vi "identify new classes.vi"(7 "existing progress bar?":bool, 8 "error in":errorcluster, 10 "force scan":bool, 11 "cache in":T1) -> (0 "error out":errorcluster, 3 "cache out":T1)   [LabVIEW 2013, in "PL_class cache.lvlib"]
uses:
  PL_class cache.lvlib
  cache definition.ctl
  cache search configuration.ctl
  cached class information.ctl
  target class metadata.ctl
  class metadata.ctl
  <vilib>/NI/Tag Bus Module Framework/root configuration/Target Types.ctl
  <vilib>/NI/Configuration Framework/class discovery singleton/class discovery singleton methods.ctl
  <vilib>/NI/Progress Bar/Controls/Update Bar Actions.ctl
  cache data.vi
  <vilib>/NI/Configuration Framework/class discovery singleton/class discovery singleton.lvlib
  <vilib>/NI/Tag Bus Module Framework/root configuration/TBM configuration.lvclass
  <vilib>/NI/Progress Bar/Progress Bar.lvlib
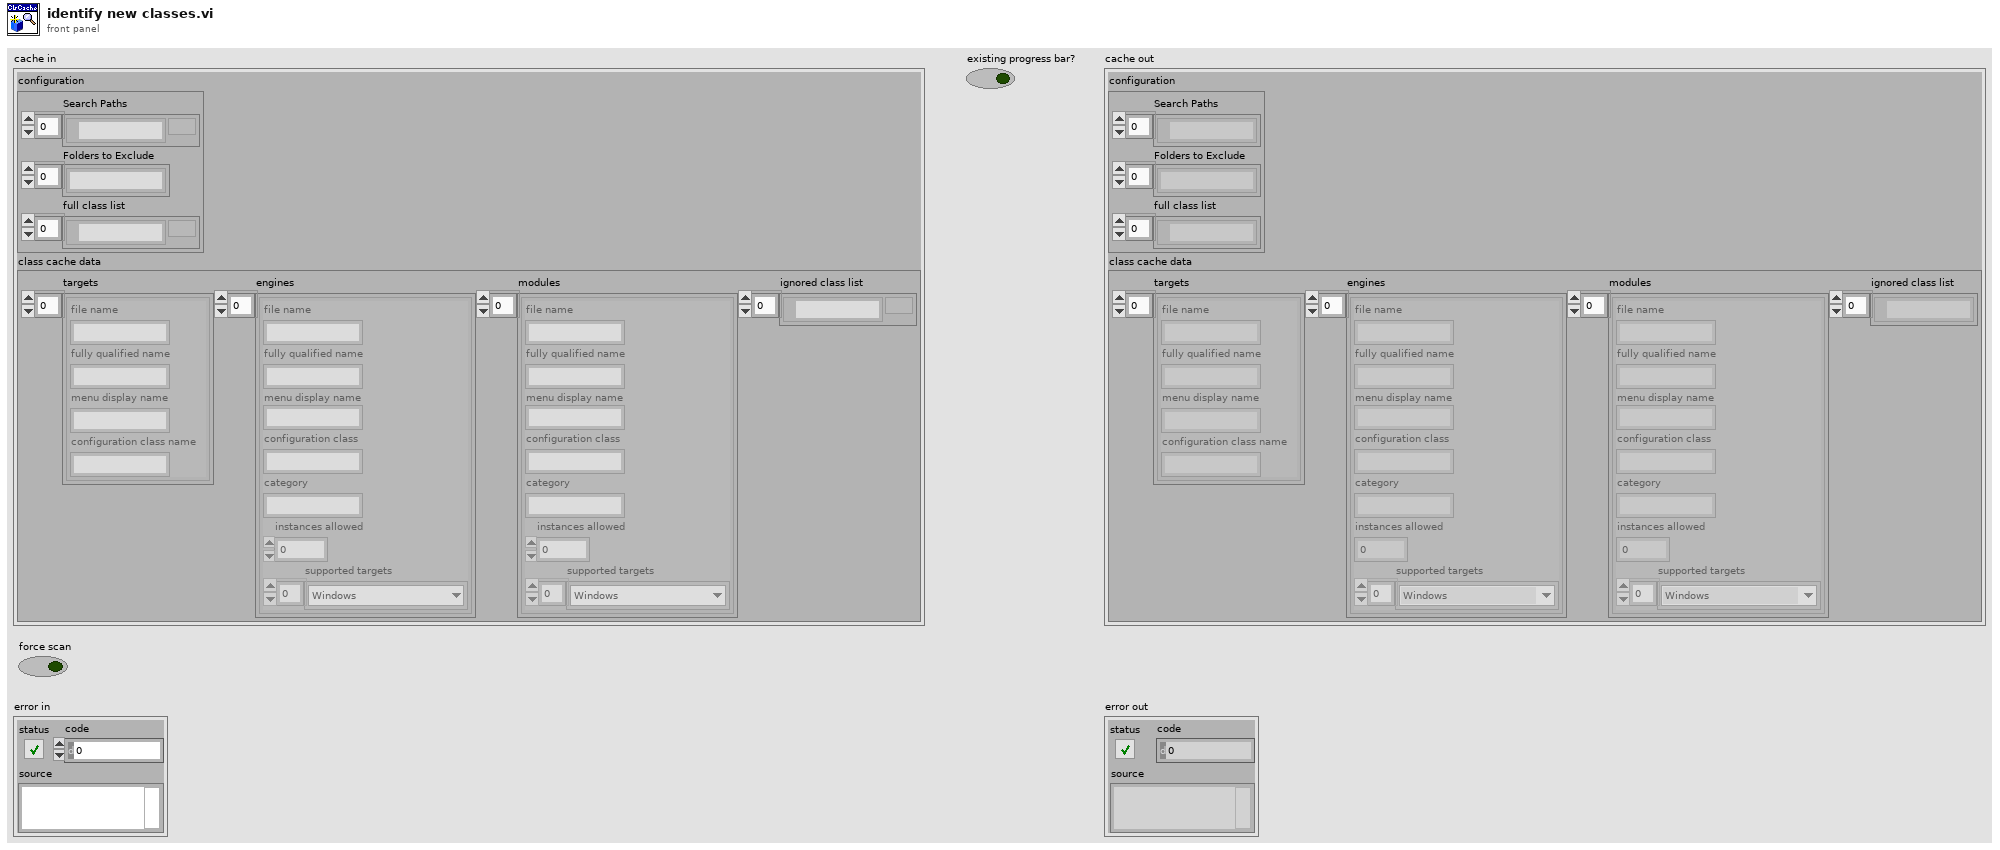
[diagram p1: front panel]
types:
  T1 = typedef "PL_class cache.lvlib/cache definition.ctl" = cluster{"configuration":T2, "class cache data":T3}
  T2 = typedef "PL_class cache.lvlib/cache search configuration.ctl" = cluster{"Search Paths":path[], "Folders to Exclude":string[], "full class list":path[]}
  T3 = typedef "PL_class cache.lvlib/cached class information.ctl" = cluster{"targets":T4[], "engines":T5[], "modules":T5[], "ignored class list":path[]}
  T4 = typedef "PL_class cache.lvlib/target class metadata.ctl" = cluster{"file name":string, "fully qualified name":string, "menu display name":string, "configuration class name":string}
  T5 = typedef "PL_class cache.lvlib/class metadata.ctl" = cluster{"file name":string, "fully qualified name":string, "menu display name":string, "configuration class":string, "category":string, "instances allowed":i32, "supported targets":T6[]}
  T6 = typedef "TBM configuration.lvclass/Target Types.ctl" = enum16{"Windows", "Mac", "Linux", "Linux RT ARM", "VxWorks", "Pharlap", "Other", "Linux RT x64"}
  T7 = typedef "class discovery singleton.lvlib/class discovery singleton methods.ctl" = enum16{"add search paths", "load class by name", "list available classes", "get class path", "delete cache"}
  T8 = typedef "Progress Bar.lvlib/Update Bar Actions.ctl" = enum16{"Add To Existing", "Set to Value"}
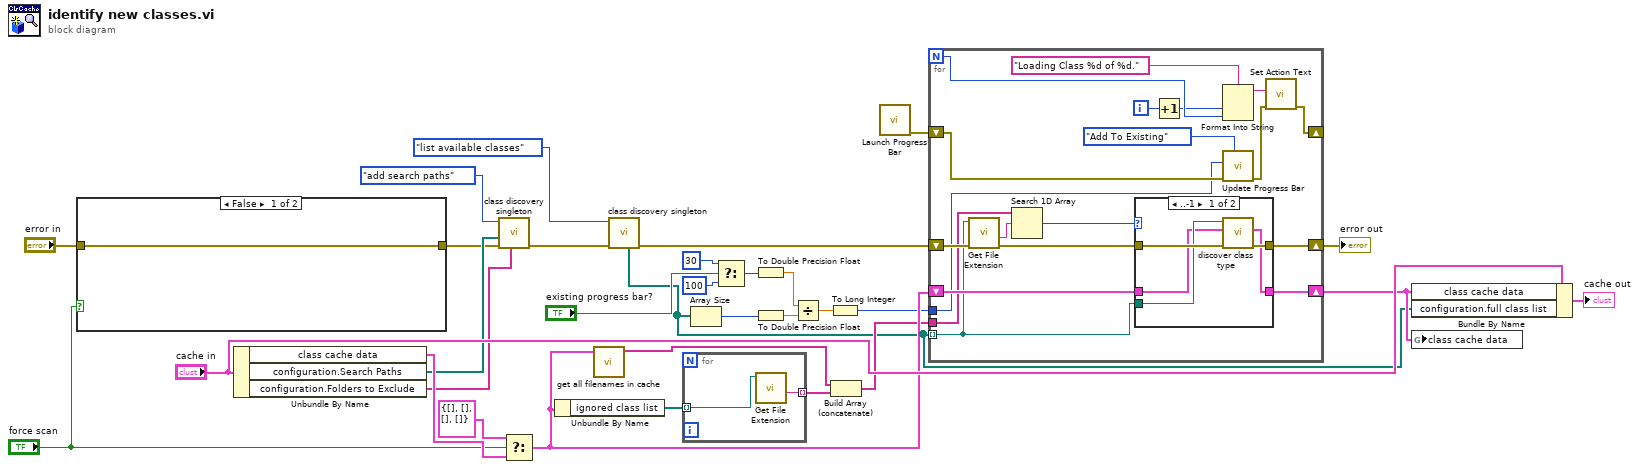
[diagram p0: block diagram]
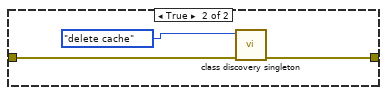
[diagram p2: hidden frame]
diagram:
  n1 = case shown="False" "force scan" {
    tunnel: "error in" -> [w32 w34]
    tunnel: [w32 w33] -> w13
    frame False {
    }
    frame True {
      n2 = call <vilib>:"class discovery singleton.vi"("error in"=w34, "method"=class_discovery_singleton_methods."delete cache") -> ("error out"=w33:errorcluster)  [unwired: 6 in, 3 out]
    }
  }
  n3 = Unbundle By Name("cache in") -> ("class cache data"=w28:T3, "configuration.Search Paths"=w26:path[], "configuration.Folders to Exclude"=w25:string[])
  n4 = call <vilib>:"class discovery singleton.vi"("Folders to Exclude"=w25, "error in"=w13, "Plugin Search Paths"=w26, "method"=class_discovery_singleton_methods."add search paths") -> ("error out"=w24:errorcluster)  [unwired: 4 in, 3 out]
  n5 = Select(t=T3 {"targets"=[], "engines"=[], "modules"=[], "ignored class list"=[]} ("class cache data"), s="force scan", f=w28) -> (s? t:f=w18:T3)
  n6 = Unbundle By Name(w18) -> ("ignored class list"=w17:path[])
  n7 = call "get all filenames in cache.vi"("class cache data"=w18) -> ("Array"=w20:string[])  [unwired: 10 in]
  n8 = call <vilib>:"class discovery singleton.vi"("error in"=w24, "method"=class_discovery_singleton_methods."list available classes") -> ("error out"=w23:errorcluster, "discovered classes"=w7:path[])  [unwired: 6 in, 2 out]
  n9 = for {
    tunnel: [w37] -> w15 mode=indexing
    tunnel: w17 -> [w36] mode=indexing
    n10 = call <vilib>:"Get File Extension.vi"("file"=w36) -> ("filename without extension"=w37:string)  [unwired: 7 in, 3 out]
  }
  n11 = Array Size(array=w7) -> (size(s)=w2:i32)
  n12 = Select(t=30, s="existing progress bar?", f=100 ("x")) -> (s? t:f=w4:i32)
  n13 = To Double Precision Float(number=w4) -> (double precision float=w3:dbl)
  n14 = To Double Precision Float(number=w2) -> (double precision float=w1:dbl)
  n15 = Divide(x=w3, y=w1) -> (x/y=w6:dbl)
  n16 = To Long Integer(number=w6) -> (32bit integer=w5:i32)
  n17 = Build Array (concatenate)(w20, w15) -> (w16:string[])
  n18 = call <vilib>:"Launch Progress Bar.vi"() -> ("error out"=w11:errorcluster)  [unwired: 10 in, 1 out]
  n19 = for {
    N -> [w41]
    tunnel: w7 -> [w51] mode=indexing
    shift-right: [w56] -> w19
    shift-left: w18 -> [w55]
    shift-right: [w54] -> w29
    shift-left: w23 -> [w53]
    tunnel: w16 -> [w50]
    shift-right: [w42] -> _
    shift-left: w11 -> [w43]
    tunnel: w5 -> [w38]
    i -> [w39]
    n20 = call <vilib>:"Get File Extension.vi"("error in (no error)"=w53, "file"=w51) -> ("error out"=w52:errorcluster, "filename without extension"=w49:string)  [unwired: 6 in, 2 out]
    n21 = Search 1D Array(1D array=w50, element=w49) -> (index of element=w48:i32)  [unwired: 1 in]
    n22 = case shown="..-1" w48 {
      tunnel: [w57 w63] -> w56
      tunnel: w55 -> [w58 w63]
      tunnel: [w59 w62] -> w54
      tunnel: w52 -> [w61 w62]
      tunnel: w51 -> [w60 _]
      frame ..-1 {
        n23 = call "discover class type.vi"("error in"=w61, "class cache data in"=w58, "Path"=w60) -> ("error out"=w59:errorcluster, "class cache data out"=w57:T3)  [unwired: 7 in]
      }
      frame 0.. {
      }
    }
    n24 = Increment(x=w39) -> (x+1=w40:i32)
    n25 = Format Into String(format string="Loading Class %d of %d.", w40, w41) -> (resulting string=w45:string)  [unwired: 2 in, 1 out]
    n26 = call <vilib>:"Update Progress Bar.vi"("Action"=Update_Bar_Actions."Add To Existing", "error in (no error)"=w43, "Value"=w38) -> ("error out"=w46:errorcluster)  [unwired: 8 in]
    n27 = call <vilib>:"Set Action Text.vi"("error in (no error)"=w46, "Action Text"=w45) -> ("error out"=w42:errorcluster)  [unwired: 9 in]
  }
  "error out" <- w29
  n28 = Bundle By Name(cluster="cache in", "class cache data"=w19, "configuration.full class list"=w7) -> (→"cache out":T1)
  n29 = global write "cache data.vi" "class cache data"(w19) -> ()
